vi "SPCNT_Read.vi"(11 "N per point":i32) -> (1 "x/y":dbl, 2 "Array":string[](array[string]))   [LabVIEW 2025]
panel:
  out "Count":i32
  in  "x":dbl
  in  "Tset setting":dbl
  in  "Boolean":bool
  out "output array":string[](array[string])
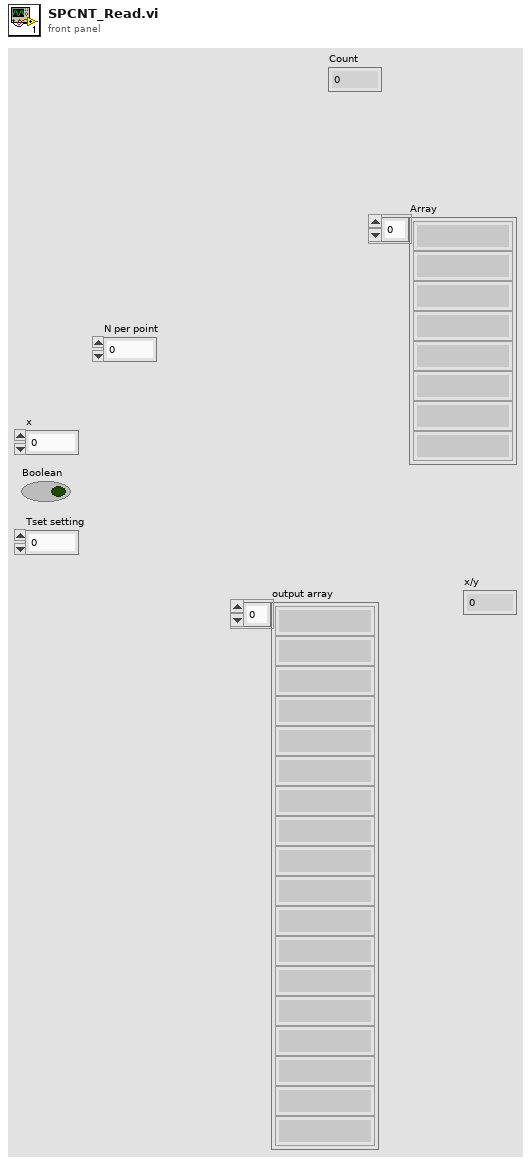
[diagram p1: front panel]
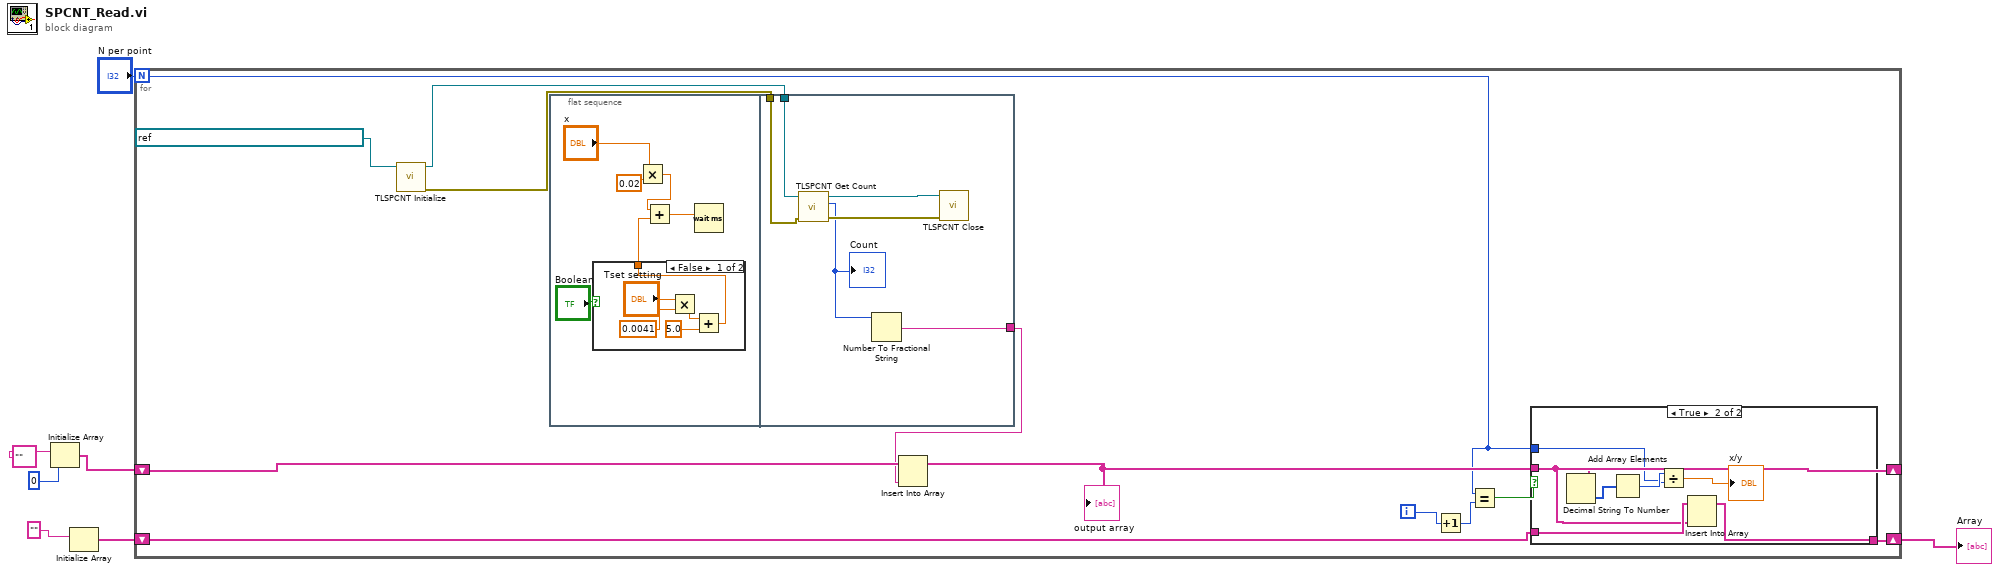
[diagram p0: block diagram]
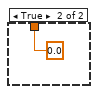
[diagram p3: hidden frame]
diagram:
  n1 = Initialize Array("", 0 ("dimension size")) -> (w6:string[])
  n2 = Initialize Array("") -> (w2:string[])  [unwired: 1 in]
  n3 = for {
    N: "N per point" -> [w16]
    shift-right: [w17] -> _
    shift-left: w6 -> [w19]
    shift-right: [w13] -> w1
    shift-left: w2 -> [w12]
    i -> [w14]
    n4 = call <instrlib>:"TLSPCNT Initialize.vi"("resource name"=refnum<visa-resource-name> "USB0::0x1313::0x8091::M01324969::INSTR" ("VISA resource name")) -> ("error out"=w8:errorcluster, "instrument handle out"=w9:refnum<visa-resource-name>)  [unwired: 9 in]
    n5 = flat-sequence {
      tunnel: [w41] -> w11
      tunnel: w9 -> [w40]
      tunnel: w8 -> [w39]
      frame #0 {
        n6 = case shown="False" "Boolean" {
          tunnel: [w33 0.0] -> w28
          frame False {
            n7 = Multiply(x="Tset setting", y=0.0041) -> (x*y=w35:dbl)
            n8 = Add(x=w35, y=5.0) -> (x+y=w33:dbl)
          }
          frame True {
          }
        }
        n9 = Multiply(x="x", y=0.02) -> (x*y=w29:dbl)
        n10 = Add(x=w29, y=w28) -> (x+y=w30:dbl)
        n11 = Wait (ms)(milliseconds to wait=w30) -> ()  [unwired: 1 out]
      }
      frame #1 {
        n12 = call <instrlib>:"TLSPCNT Get Count.vi"("error in (no error)"=w39, "instrument handle"=w40) -> ("error out"=w44:errorcluster, "Count"=w42:i32, "instrument handle out"=w43:refnum<visa-resource-name>)  [unwired: 7 in]
        "Count" <- w42
        n13 = Number To Fractional String(number=w42) -> (F-format string=w41:string)  [unwired: 3 in]
        n14 = call <instrlib>:"TLSPCNT Close.vi"("error in (no error)"=w44, "instrument handle"=w43) -> ()  [unwired: 9 in, 1 out]
      }
    }
    n15 = Insert Into Array(array=w19, new element=w11) -> (w17:string[])  [unwired: 1 in]
    "output array" <- w17
    n16 = Increment(x=w14) -> (x+1=w15:i32)
    n17 = Equal?(x=w16, y=w15) -> (x = y?=w18:bool)
    n18 = case shown="True" w18 {
      tunnel: w17 -> [_ w21]
      tunnel: w16 -> [_ w24]
      tunnel: [_ w20] -> w13
      tunnel: w12 -> [_ w22]
      frame False {
      }
      frame True {
        n19 = Decimal String To Number(string=w21) -> (number=w26:i32[])  [unwired: 2 in, 1 out]
        n20 = Add Array Elements(numeric array=w26) -> (sum=w25:i32)
        n21 = Divide(x=w25, y=w24) -> (x/y=→"x/y":dbl)
        n22 = Insert Into Array(array=w22, new element=w21) -> (w20:string[])  [unwired: 1 in]
      }
    }
  }
  "Array" <- w1
